vi "RestartVI.vi"(0 "Application Ref in":refnum<vi>, 5 "VI in":refnum<vi>, 11 "error in (no error)":errorcluster) -> (4 "Application Ref out":refnum<vi>, 6 "VI out":refnum<vi>, 15 "error out":errorcluster)   [LabVIEW 2016, in "CarWashTest.lvlib"]
doc: "Restart the main VI"
uses:
  CarWashTest.lvlib
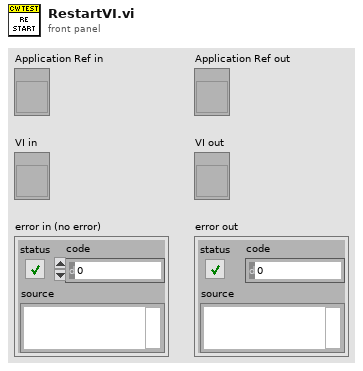
[diagram p1: front panel]
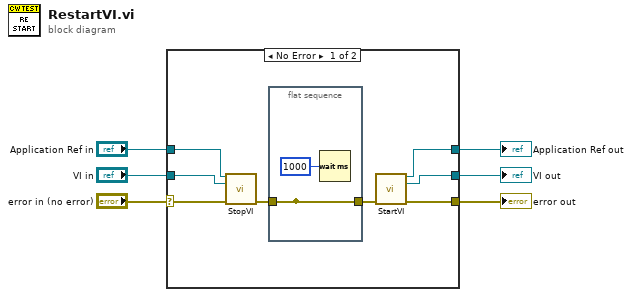
[diagram p0: block diagram]
diagram:
  n1 = case shown="No Error" "error in (no error)" {
    selector: "error in (no error)" -> [w9 w19]
    tunnel: [w14 w18] -> w6
    tunnel: [w13 w17] -> w5
    tunnel: "VI in" -> [w12 w18]
    tunnel: "Application Ref in" -> [w11 w17]
    tunnel: [w10 w19] -> w2
    frame No Error {
      n2 = call "StopVI.vi"("Application Ref in"=w11, "VI in"=w12, "error in (no error)"=w9) -> ("error out"=w8:errorcluster)  [unwired: 12 in]
      n3 = flat-sequence {
        tunnel: [w15] -> _
        tunnel: w8 -> [w15]
        tunnel: [w15] -> w7
        frame #0 {
          n4 = Wait (ms)(milliseconds to wait=u32 1000) -> ()  [unwired: 1 out]
        }
      }
      n5 = call "StartVI.vi"("error in"=w7) -> ("Application Ref out"=w13:refnum<vi>, "VI Reference"=w14:refnum<vi>, "error out"=w10:errorcluster)  [unwired: 12 in]
    }
    frame Error {
    }
  }
  "VI out" <- w6
  "Application Ref out" <- w5
  "error out" <- w2
